vi "~ct - Get 2 numeric args (poly).vi"(7 "InstanceRef":T5, 11 "args list":T6[](array[typedef])) -> (0 "poly":T1(ring), 1 "CDB ?":bool, 2 "CDB arguments":T3 {"Right Scalar" format="%.2f"; "Right 2D" format="%.2f"; "Left Scalar" format="%.2f"; "Left 2D" format="%.2f"}, 3 "DBL arguments":T4 {"Right Scalar" format="%.2f"; "Right 2D" format="%.2f"; "Left Scalar" format="%.2f"; "Left 2D" format="%.2f"}, 4 "error out":bool, 6 "type of result":T2)   [LabVIEW 2021]
doc: "::: CalcExpress Toolkit :::\nCopyright (c) 2000-2026 Konstantin Shifershteyn. All rights reserved."
uses:
  cetypes.llb/CalcExpress Function Argument Info.ctl
  cetypes.llb/CalcExpress Instance RefNum.ctl
  cetypes.llb/CalcExpress Data Type.ctl
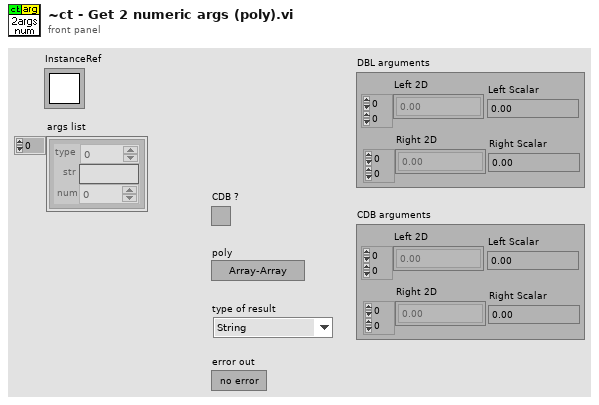
[diagram p1: front panel]
types:
  T1 = enum16{"Array-Array", "Array-Scalar", "Scalar-Array", "Scalar-Scalar"}
  T2 = typedef "CalcExpress Data Type.ctl" = enum32{"String", "DBL Number", "identifier", "1D Array of DBL", "2D Array of DBL", "CDB Number", "1D Array of CDB", "2D Array of CDB", "1D Array of String", "2D Array of String", "Unknown data type"}
  T3 = cluster{"Left 2D":cdb[][], "Left Scalar":cdb, "Right 2D":cdb[][], "Right Scalar":cdb}
  T4 = cluster{"Left 2D":dbl[][], "Left Scalar":dbl, "Right 2D":dbl[][], "Right Scalar":dbl}
  T5 = typedef "CalcExpress Instance RefNum.ctl" = refnum<k1>
  T6 = typedef "CalcExpress Function Argument Info.ctl" = cluster{"type":u32, "str":string, "num":dbl}
  T7 = enum16{"DBL scalar", "CDB scalar", "DBL array", "CDB array", "ERROR"}
  T8 = enum32{"String", "DBL Number", "identifier", "1D Array of DBL", "2D Array of DBL", "CDB Number", "1D Array of CDB", "2D Array of CDB", "1D Array of String", "2D Array of String", "Unknown data type"}
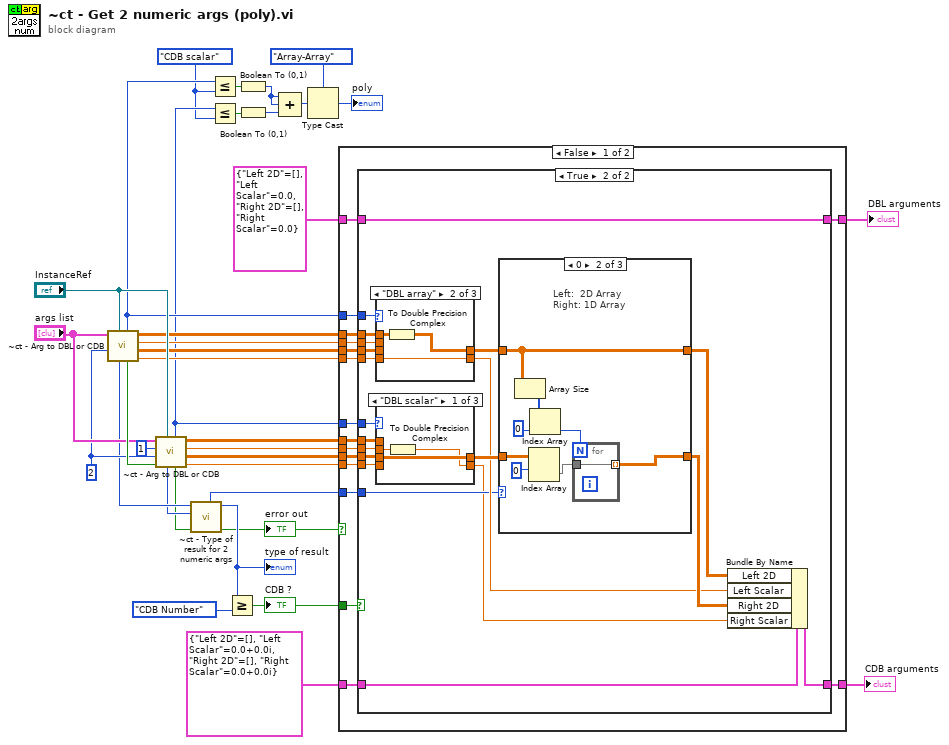
[diagram p0: block diagram]
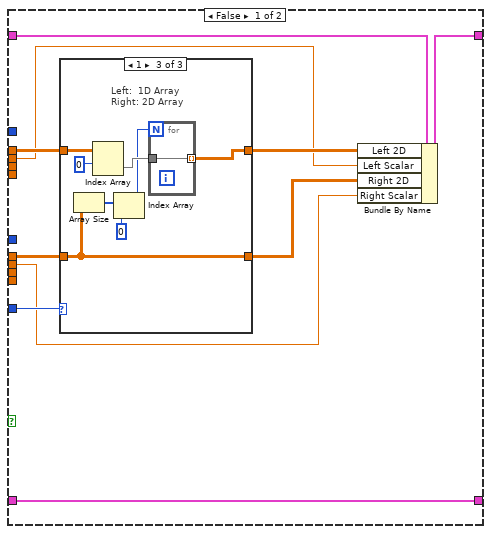
[diagram p2: hidden frame]
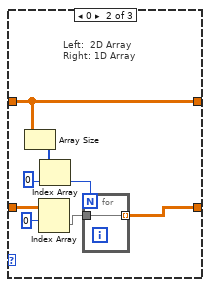
[diagram p4: hidden frame]
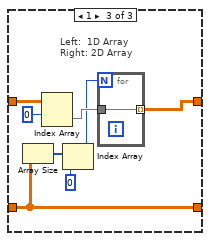
[diagram p6: hidden frame]
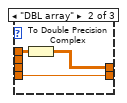
[diagram p7: hidden frame]
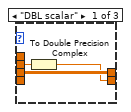
[diagram p9: hidden frame]
diagram:
  w2 = T7."CDB scalar" ("category")
  w31 = 2 ("max args")
  n1 = call "~ct - Arg to DBL or CDB.vi"("InstanceRef"="InstanceRef", "max args"=w31, "args list"="args list") -> ("CDB"=w27:cdb, "2D CDB"=w28:cdb[][], "DBL"=w29:dbl, "2D DBL"=w30:dbl[][], "error out"=w35:bool, "category"=w10:T7, "arg type"=w21:T2)  [unwired: 2 in]
  n2 = call "~ct - Arg to DBL or CDB.vi"("InstanceRef"="InstanceRef", "error in"=w35, "max args"=w31, "arg index"=1, "args list"="args list") -> ("CDB"=w23:cdb, "2D CDB"=w24:cdb[][], "DBL"=w25:dbl, "2D DBL"=w26:dbl[][], "error out"=w19:bool, "category"=w9:T7, "arg type"=w20:T2)
  n3 = call "~ct - Type of result for 2 numeric args.vi"("error in"=w19, "type of right"=w20, "type of left"=w21) -> ("error out"=w11:bool, "type of result"=w13:T2, "1D-2D sign"=w18:i32)  [unwired: 4 in]
  "type of result" <- w13
  "error out" <- w11
  n4 = Less Or Equal?(x=w10, y=w2) -> (x <= y?=w4:bool)
  n5 = Less Or Equal?(x=w9, y=w2) -> (x <= y?=w3:bool)
  n6 = Greater Or Equal?(x=w13, y=T8."CDB Number") -> (x >= y?=w12:bool)
  "CDB ?" <- w12
  n7 = Boolean To (0,1)(Boolean=w4) -> (0, 1=w8:i16)
  n8 = Boolean To (0,1)(Boolean=w3) -> (0, 1=w7:i16)
  n9 = Compound Arithmetic op=ADD(w8, w8, w7) -> (w6:i16)
  n10 = Type Cast(type=T1."Array-Array" ("poly"), x=w6) -> (*(type *) &x=→"poly":T1)
  n11 = case shown="False" w11 {
    tunnel: w12 -> [w51 _]
    tunnel: w10 -> [w50 _]
    tunnel: w30 -> [w49 _]
    tunnel: w29 -> [w48 _]
    tunnel: w28 -> [w47 _]
    tunnel: w27 -> [w46 _]
    tunnel: w26 -> [w45 _]
    tunnel: w25 -> [w44 _]
    tunnel: w24 -> [w43 _]
    tunnel: w23 -> [w42 _]
    tunnel: w18 -> [w41 _]
    tunnel: [w40 w139] -> w17
    tunnel: w9 -> [w39 _]
    tunnel: T4 {"Left 2D"=[], "Left Scalar"=0.0, "Right 2D"=[], "Right Scalar"=0.0} ("DBL arguments") -> [w38 w139]
    tunnel: [w37 w138] -> w15
    tunnel: T3 {"Left 2D"=[], "Left Scalar"=0.0+0.0i, "Right 2D"=[], "Right Scalar"=0.0+0.0i} ("CDB arguments") -> [w36 w138]
    frame False {
      n12 = case shown="True" w51 {
        tunnel: w50 -> [_ w101]
        tunnel: w49 -> [w58 w100]
        tunnel: w48 -> [w56 w99]
        tunnel: w47 -> [_ w98]
        tunnel: w46 -> [_ w97]
        tunnel: w45 -> [w61 w96]
        tunnel: w44 -> [w55 w95]
        tunnel: w43 -> [_ w94]
        tunnel: w42 -> [_ w93]
        tunnel: w41 -> [w60 w83]
        tunnel: [w54 w91] -> w40
        tunnel: w39 -> [_ w92]
        tunnel: w38 -> [w53 w91]
        tunnel: [w52 w88] -> w37
        tunnel: w36 -> [w52 w87]
        frame False {
          n13 = case shown="1" w60 {
            tunnel: w58 -> [w63 w69 w76]
            tunnel: w61 -> [w62 w67 w78]
            tunnel: [w62 w64 w78] -> w57
            tunnel: [w63 w69 w73] -> w59
            frame -1, Default {
            }
            frame 0 {
              # "Left:  2D Array\nRight: 1D Array"
              n14 = Array Size(array=w69) -> (size(s)=w71:i32[])
              n15 = Index Array(array=w67, index (row)=0) -> (element=w68:dbl[])  [unwired: 1 in]
              n16 = Index Array(array=w71, index=0) -> (element=w66:i32)
              n17 = for {
                N: w66 -> [_]
                tunnel: w68 -> [w72]
                tunnel: [w72] -> w64 mode=indexing
              }
            }
            frame 1 {
              # "Left:  1D Array\nRight: 2D Array"
              n18 = Array Size(array=w78) -> (size(s)=w80:i32[])
              n19 = Index Array(array=w76, index (row)=0) -> (element=w77:dbl[])  [unwired: 1 in]
              n20 = Index Array(array=w80, index=0) -> (element=w75:i32)
              n21 = for {
                N: w75 -> [_]
                tunnel: w77 -> [w81]
                tunnel: [w81] -> w73 mode=indexing
              }
            }
          }
          n22 = Bundle By Name(cluster=w53, "Left 2D"=w59, "Left Scalar"=w56, "Right 2D"=w57, "Right Scalar"=w55) -> (w54:T4)
        }
        frame True {
          n23 = case shown="\"DBL array\"" w101 {
            tunnel: w100 -> [_ w134 _]
            tunnel: w99 -> [w131 _ _]
            tunnel: w98 -> [w132 _ w136]
            tunnel: w97 -> [_ w135 w137]
            tunnel: [w130 w135 w137] -> w84
            tunnel: [w132 w133 w136] -> w90
            frame "DBL scalar" {
              n24 = To Double Precision Complex(1:w131) -> (0:w130:cdb)
            }
            frame "DBL array" {
              n25 = To Double Precision Complex(1:w134) -> (0:w133:cdb[][])
            }
            frame Default {
            }
          }
          n26 = case shown="\"DBL scalar\"" w92 {
            tunnel: w96 -> [_ w126 _]
            tunnel: w95 -> [w123 _ _]
            tunnel: w94 -> [w124 _ w128]
            tunnel: w93 -> [_ w127 w129]
            tunnel: [w122 w127 w129] -> w82
            tunnel: [w124 w125 w128] -> w89
            frame "DBL scalar" {
              n27 = To Double Precision Complex(1:w123) -> (0:w122:cdb)
            }
            frame "DBL array" {
              n28 = To Double Precision Complex(1:w126) -> (0:w125:cdb[][])
            }
            frame Default {
            }
          }
          n29 = case shown="0" w83 {
            tunnel: w90 -> [w103 w109 w116]
            tunnel: w89 -> [w102 w107 w118]
            tunnel: [w102 w104 w118] -> w85
            tunnel: [w103 w109 w113] -> w86
            frame -1, Default {
            }
            frame 0 {
              # "Left:  2D Array\nRight: 1D Array"
              n30 = Array Size(array=w109) -> (size(s)=w111:i32[])
              n31 = Index Array(array=w107, index (row)=0) -> (element=w108:cdb[])  [unwired: 1 in]
              n32 = Index Array(array=w111, index=0) -> (element=w106:i32)
              n33 = for {
                N: w106 -> [_]
                tunnel: w108 -> [w112]
                tunnel: [w112] -> w104 mode=indexing
              }
            }
            frame 1 {
              # "Left:  1D Array\nRight: 2D Array"
              n34 = Array Size(array=w118) -> (size(s)=w120:i32[])
              n35 = Index Array(array=w116, index (row)=0) -> (element=w117:cdb[])  [unwired: 1 in]
              n36 = Index Array(array=w120, index=0) -> (element=w115:i32)
              n37 = for {
                N: w115 -> [_]
                tunnel: w117 -> [w121]
                tunnel: [w121] -> w113 mode=indexing
              }
            }
          }
          n38 = Bundle By Name(cluster=w87, "Left 2D"=w86, "Left Scalar"=w84, "Right 2D"=w85, "Right Scalar"=w82) -> (w88:T3)
        }
      }
    }
    frame True {
    }
  }
  "DBL arguments" <- w17
  "CDB arguments" <- w15
